vi "I Exist.vi"(8 "error in (no error)":errorcluster, 11 "Guardian in":refnum<class "Guardian.lvclass">) -> (0 "error out":errorcluster, 3 "Guardian out":refnum<class "Guardian.lvclass">)   [LabVIEW 2020, in "TALOS.lvlib" / "Guardian.lvlib" / "Guardian.lvclass"]
uses:
  Guardian.lvclass
  C:/Users/marco/Documents/GitHub_Lab/TALOS/talos/Ancestor/Ancestor/Ancestor.lvclass
  Ancestor/Ancestor/Ancestor.lvclass/Ancestor.ctl
  Guardian.lvclass/Guardian.ctl
  Classes/Guardian List/Guardian List.lvclass
  Ancestor/Ancestor/Ancestor.lvclass
  TALOS.lvlib
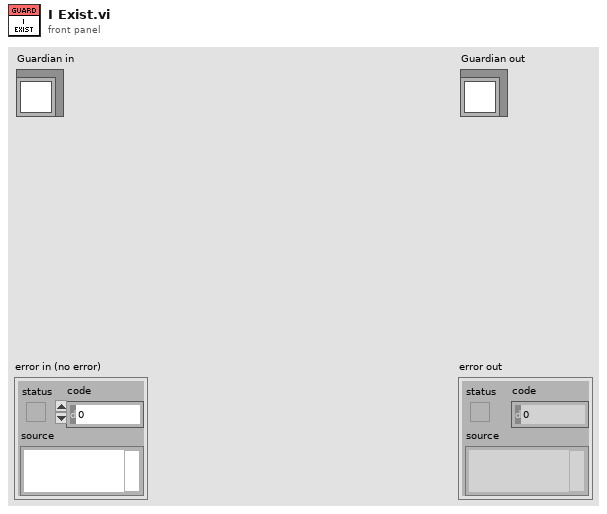
[diagram p1: front panel]
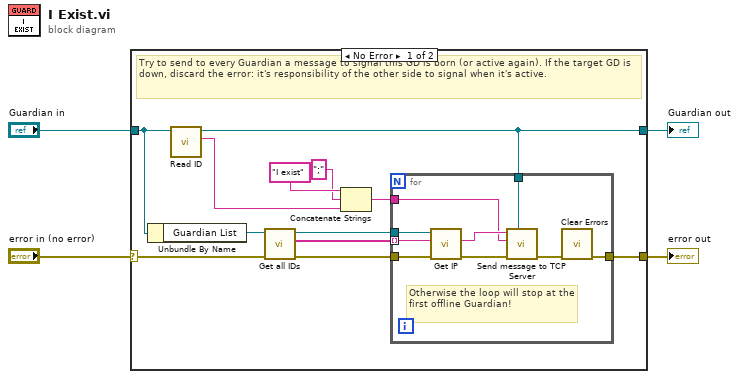
[diagram p0: block diagram]
diagram:
  n1 = case shown="No Error" "error in (no error)" {
    selector: "error in (no error)" -> [w12 w27]
    tunnel: [w9 w27] -> w3
    tunnel: [w7 w26] -> w1
    tunnel: "Guardian in" -> [w10 w26]
    frame No Error {
      # "Try to send to every Guardian a message to signal this GD is born (or active again). If the target GD is down, discard the error: it's responsibility of the other side to signal when it's active."
      n2 = Unbundle By Name(w10) -> ("Guardian List"=w15:refnum<class "Guardian List.lvclass">)
      n3 = call "Read ID.vi"("Ancestor in"=w10) -> ("ID"=w16:string, "Ancestor out"=w7:refnum<class "Guardian.lvclass">)  [unwired: 8 in, 1 out]
      n4 = call-dynamic "Get all IDs.vi"("error in (no error)"=w12, "Guardian List in"=w15) -> ("error out"=w13:errorcluster, "All IDs"=w14:string[], "Guardian List out"=w8:refnum<class "Guardian List.lvclass">)  [unwired: 7 in]
      n5 = Concatenate Strings("I exist" ("Message"), ";" ("string"), w16) -> (w5:string)
      n6 = for {
        tunnel: w8 -> [w24]
        tunnel: w13 -> [w23]
        tunnel: [w19] -> w9
        tunnel: w14 -> [w22] mode=indexing
        tunnel: w5 -> [w17]
        tunnel: w7 -> [w20]
        # "Otherwise the loop will stop at the first offline Guardian!"
        n7 = call-dynamic "Get IP.vi"("error in (no error)"=w23, "ID"=w22, "Guardian List in"=w24) -> ("error out"=w25:errorcluster, "IP"=w18:string)  [unwired: 6 in, 1 out]
        n8 = call "Send message to TCP Server.vi"("LabVIEW Object"=w20, "error in (no error)"=w25, "String"=w17, "IP"=w18) -> ("error out"=w21:errorcluster)  [unwired: 7 in]
        n9 = call <vilib>:"Clear Errors.vi"("error in (no error)"=w21) -> ("error out"=w19:errorcluster)  [unwired: 5 in, 1 out]
      }
    }
    frame Error {
    }
  }
  "error out" <- w3
  "Guardian out" <- w1
